vi "Initialise.vi"(6 "Tag Root":string, 8 "error in (no error)":errorcluster, 9 "Channel":refnum<class "Abs_Value.lvclass">[](array[class]), 10 "VISA resource name":refnum<visa-resource-name>, 11 "CTI_Bus in":refnum<class "CTI_Bus.lvclass">) -> (0 "error out":errorcluster, 3 "CTI_Bus out":refnum<class "CTI_Bus.lvclass">)   [LabVIEW 2021, in "CTI_Bus.lvclass"]
uses:
  CTI_Bus.lvclass
  C:/Program Files (x86)/National Instruments/LabVIEW 2021/vi.lib/TSA/Omni-Bus/Omni-Bus/Bus Access/Bus_Access.lvclass
  <vilib>/TSA/Abstract Data Classes/Abs_Types/Value/Abs_Value.lvclass
  C:/Program Files (x86)/National Instruments/LabVIEW 2021/vi.lib/TSA/Abstract Data Classes/Abs_Types/Type/Abs_Type.lvclass
  CTI_Bus.lvclass/CTI_Bus.ctl
  <vilib>/TSA/Omni-Bus/Omni-Bus/Bus Access/Bus_Access.lvclass/Bus_Access.ctl
  Properties/Write Channels.vi
  <vilib>/TSA/Omni-Bus/Omni-Bus/Bus Access/Properties/Write Tag Root.vi
  Properties/Write VISA resource name.vi
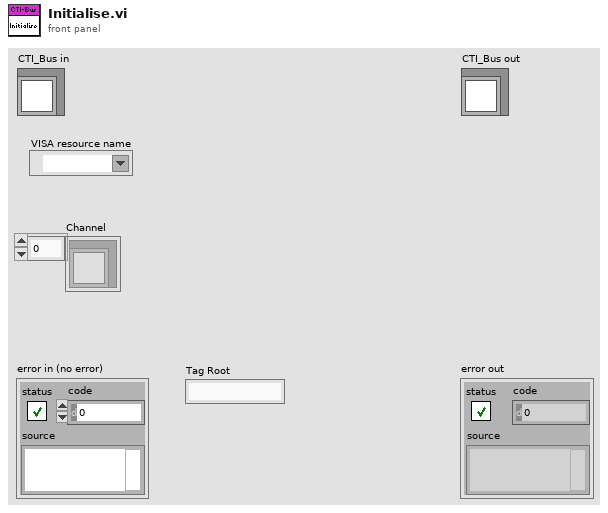
[diagram p1: front panel]
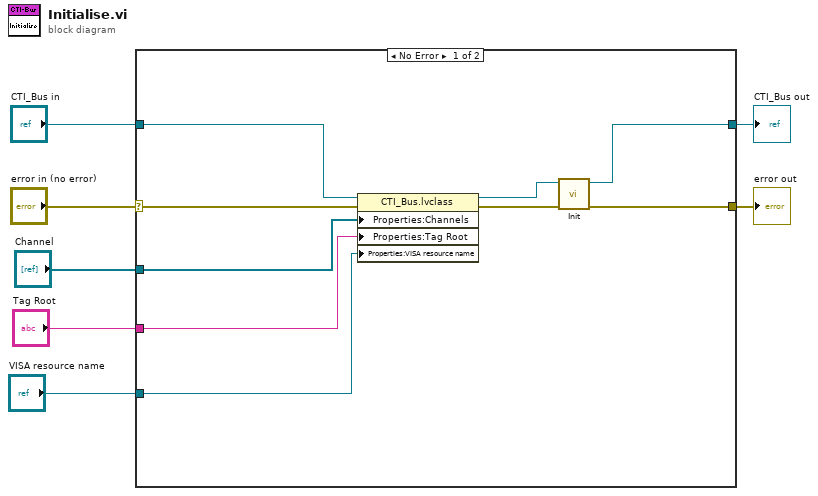
[diagram p0: block diagram]
diagram:
  n1 = case shown="No Error" "error in (no error)" {
    selector: "error in (no error)" -> [w14 w18]
    tunnel: [w16 w18] -> w6
    tunnel: [w15 w17] -> w4
    tunnel: "CTI_Bus in" -> [w12 w17]
    tunnel: "Tag Root" -> [w10 _]
    tunnel: "VISA resource name" -> [w9 _]
    tunnel: "Channel" -> [w8 _]
    frame No Error {
      n2 = property class="CTI_Bus.lvclass"(reference=w12, error in=w14, "Properties:Channels"=w8, "Properties:Tag Root"=w10, "Properties:VISA resource name"=w9) -> (reference out=w11:refnum<class "CTI_Bus.lvclass">, error out=w13:errorcluster)
      n3 = call-dynamic "Init.vi"("error in (no error)"=w13, "Data in"=w11) -> ("error out"=w16:errorcluster, "Data out"=w15:refnum<class "CTI_Bus.lvclass">)  [unwired: 8 in]
    }
    frame Error {
    }
  }
  "error out" <- w6
  "CTI_Bus out" <- w4
